vi "Own20261012_GetWhileStopIfTrue.vi"() -> ()   [LabVIEW 2024]
panel:
  out "error out":errorcluster caption="错误输出"
  out "stop_if_true":bool
  in  "while_id":u32
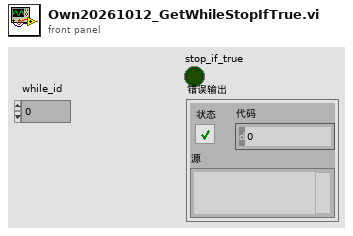
[diagram p1: front panel]
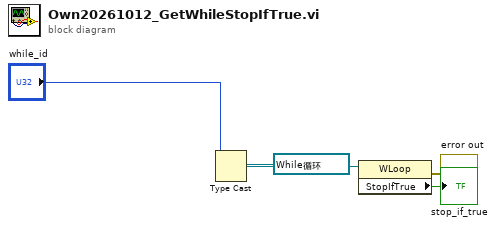
[diagram p0: block diagram]
diagram:
  n1 = Type Cast(type=refnum<vi> refnum ("引用"), x="while_id") -> (*(type *) &x=w3:refnum<vi>)
  n2 = property class="WLoop"(reference=w3) -> (error out=→"error out":errorcluster, "StopIfTrue"=→"stop_if_true":bool)  [unwired: 1 in, 1 out]
